vi "NumIntegrate_Rk4_Mat_X.vi"(5 "Func_X_Extra":refnum<vi>, 7 "PassedData":variant, 8 "dT_Seconds":dbl, 11 "X":T1) -> (0 "Error":bool, 3 "OUTPUT":T1)   [LabVIEW 2019, in "Trajectory_Library.lvlib"]
doc: "Performs 4th order Runge-Kutta integration of dx/dt = f( matrix x) for dt.\n\nInputs:\n - Func_X_Extra -- A strictly typed LabVIEW reference to a function to integrate as a function of matrix X, and the extra passed data\n - PassedData -- This is a variant that can be used to pass additional data to the function if needed. The data must be packed into the variant in the specific way expected by the function.\n - X -- X input matrix\n - dT -- Time differential in seconds\n\nOutputs:\n - OUTPUT -- The integration of dx/dt = f(x, u) for dt.\n - Error -- If TRUE, an error occured."
uses:
  Trajectory_Library.lvlib
  <vilib>/Analysis/Matrix/Datatypes/RealMatrix.ctl
  <vilib>/Analysis/Matrix/Numeric/Multiply/Multiply - RM,R.vi
  <vilib>/Analysis/Matrix/Numeric/Add/Add - RM,RM.vi
  <vilib>/Analysis/Matrix/NI_Matrix.lvlib
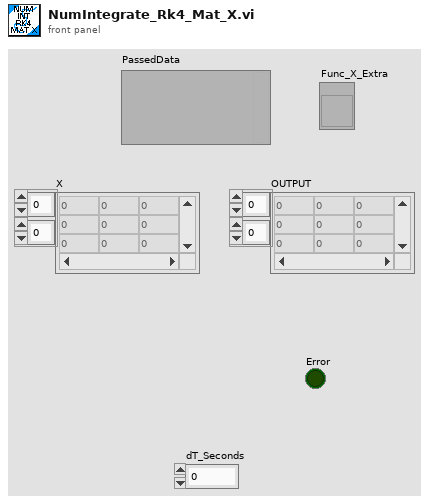
[diagram p1: front panel]
types:
  T1 = typedef "NI_Matrix.lvlib/RealMatrix.ctl" = dbl[][]
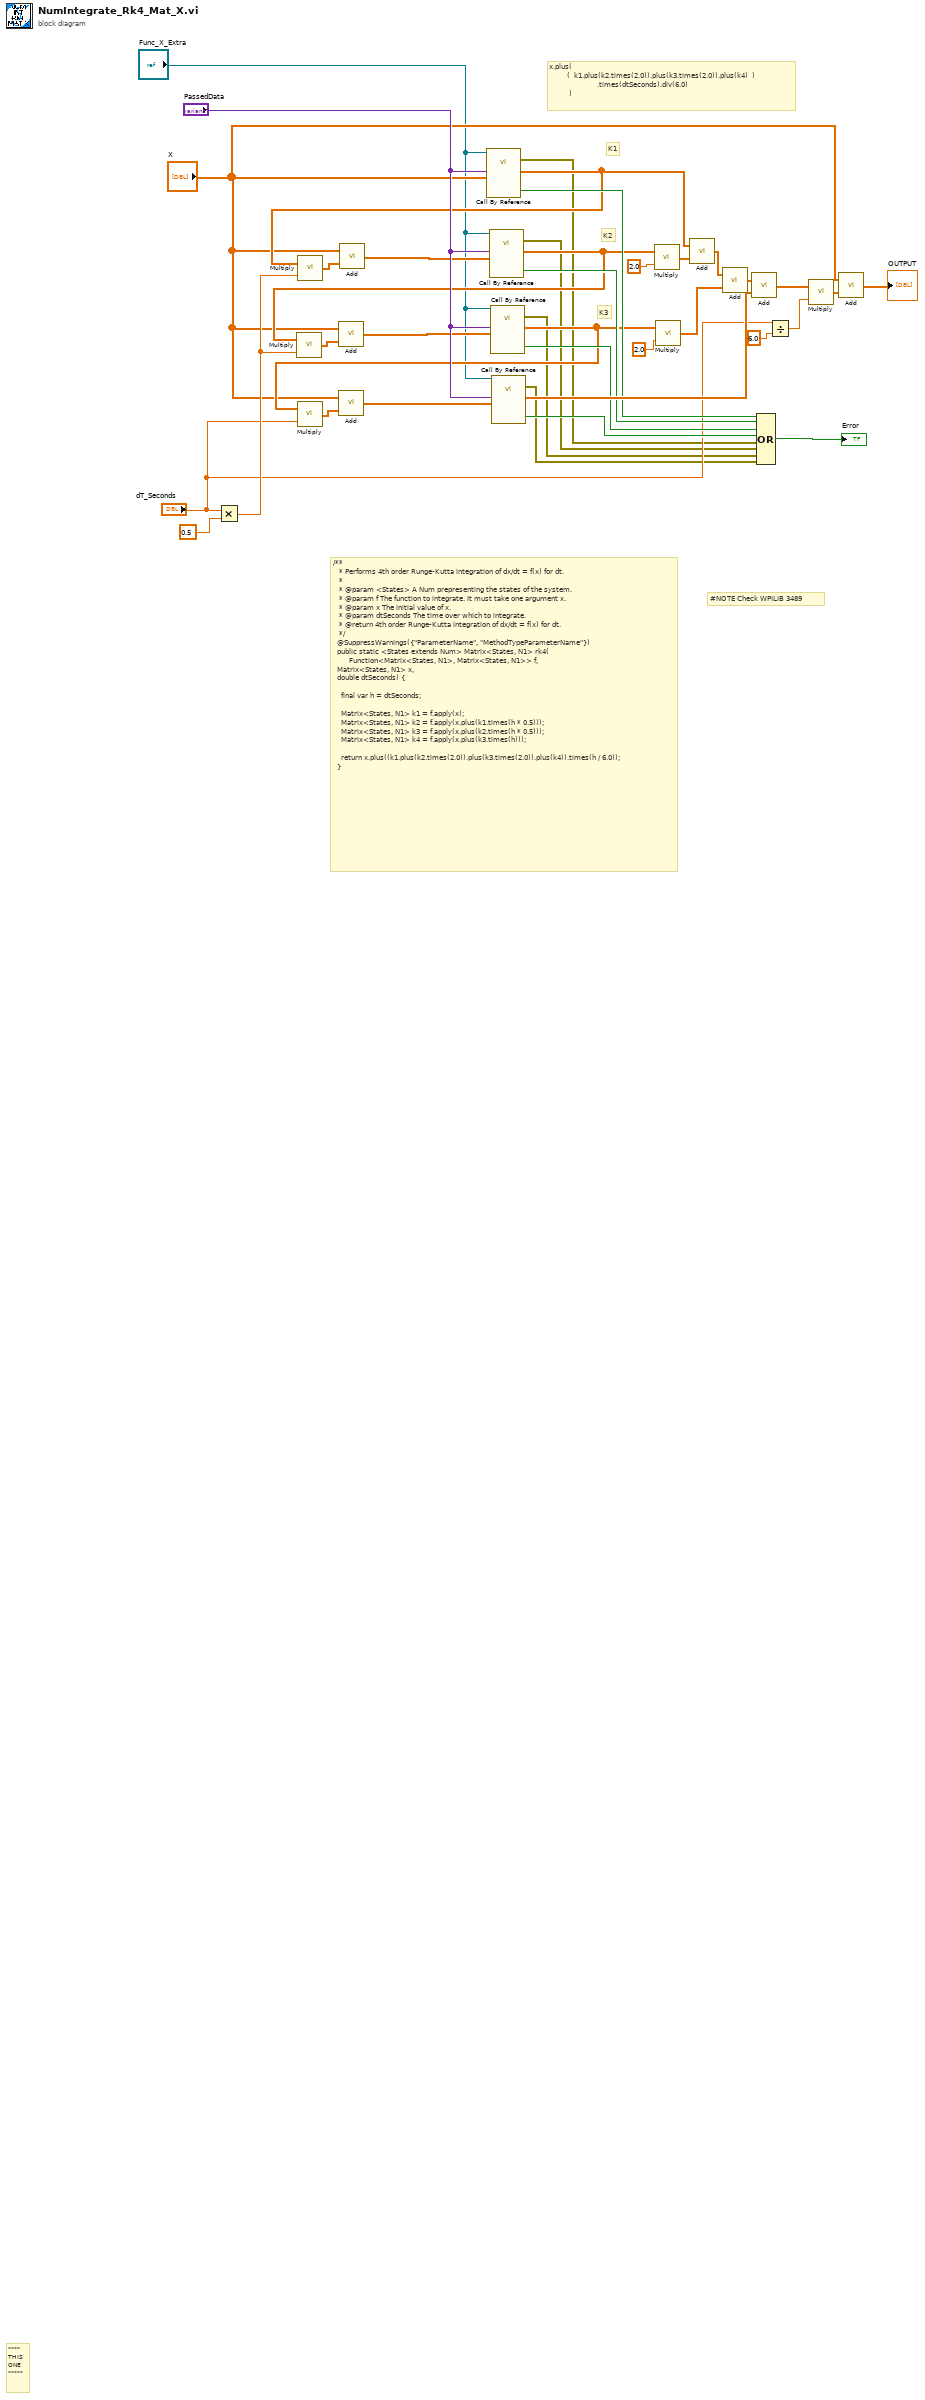
[diagram p0: block diagram]
diagram:
  # "#NOTE Check WPILIB 3489"
  # "x.plus(\n         (  k1.plus(k2.times(2.0)).plus(k3.times(2.0)).plus(k4)  )\n                        .times(dtSeconds).div(6.0)\n          )"
  # "K3"
  # "K2"
  # "K1"
  # "/**\n   * Performs 4th order Runge-Kutta integration of dx/dt = f(x) for dt.\n   *\n   * @param <States> A Num prepresenting the states of the system.\n   * @param f The function to integrate. It must take one argument x.\n   * @param x The initial value of x.\n   * @param dtSeconds The time over which to integrate.\n   * @return 4th order Runge-Kutta integration of dx/dt = f(x) for dt.\n   */\n  @SuppressWarnings({\"ParameterName\", \"MethodTypeParameterName\"})\n  public static <States extends Num> Matrix<States, N1> rk4(\n      \t\tFunction<Matrix<States, N1>, Matrix<States, N1>> f, \n\t\tMatrix<States, N1> x, \n\t\tdouble dtSeconds) {\n\n    final var h = dtSeconds;\n\n    Matrix<States, N1> k1 = f.apply(x);\n    Matrix<States, N1> k2 = f.apply(x.plus(k1.times(h * 0.5)));\n    Matrix<States, N1> k3 = f.apply(x.plus(k2.times(h * 0.5)));\n    Matrix<States, N1> k4 = f.apply(x.plus(k3.times(h)));\n\n    return x.plus((k1.plus(k2.times(2.0)).plus(k3.times(2.0)).plus(k4)).times(h / 6.0));\n  }"
  # "****\nTHIS\nONE\n*****"
  n1 = Multiply(x="dT_Seconds", y=0.5) -> (x*y=w13:dbl)
  n2 = call-by-ref "?"(reference="Func_X_Extra", "X"="X", "Variant"="PassedData") -> (error out=w5:errorcluster, "Error"=w28:bool, "NewX"=w22:T1)  [unwired: 9 in, 1 out]
  n3 = call-poly <vilib>:"Multiply.vi"("Real Scalar c"=w13, "Real Matrix A"=w22) -> ("A * c"=w21:T1)
  n4 = call-poly <vilib>:"Add.vi"("Real Matrix B"=w21, "Real Matrix A"="X") -> ("A + B"=w20:T1)
  n5 = call-by-ref "?"(reference="Func_X_Extra", "X"=w20, "Variant"="PassedData") -> (error out=w4:errorcluster, "Error"=w27:bool, "NewX"=w17:T1)  [unwired: 9 in, 1 out]
  n6 = call-poly <vilib>:"Multiply.vi"("Real Scalar c"=w13, "Real Matrix A"=w17) -> ("A * c"=w19:T1)
  n7 = call-poly <vilib>:"Add.vi"("Real Matrix B"=w19, "Real Matrix A"="X") -> ("A + B"=w18:T1)
  n8 = call-by-ref "?"(reference="Func_X_Extra", "X"=w18, "Variant"="PassedData") -> (error out=w3:errorcluster, "Error"=w26:bool, "NewX"=w14:T1)  [unwired: 9 in, 1 out]
  n9 = call-poly <vilib>:"Multiply.vi"("Real Scalar c"="dT_Seconds", "Real Matrix A"=w14) -> ("A * c"=w16:T1)
  n10 = call-poly <vilib>:"Add.vi"("Real Matrix B"=w16, "Real Matrix A"="X") -> ("A + B"=w15:T1)
  n11 = call-by-ref "?"(reference="Func_X_Extra", "X"=w15, "Variant"="PassedData") -> (error out=w2:errorcluster, "Error"=w25:bool, "NewX"=w29:T1)  [unwired: 9 in, 1 out]
  n12 = call-poly <vilib>:"Multiply.vi"("Real Scalar c"=2.0, "Real Matrix A"=w17) -> ("A * c"=w33:T1)
  n13 = call-poly <vilib>:"Multiply.vi"("Real Scalar c"=2.0, "Real Matrix A"=w14) -> ("A * c"=w31:T1)
  n14 = call-poly <vilib>:"Add.vi"("Real Matrix B"=w33, "Real Matrix A"=w22) -> ("A + B"=w32:T1)
  n15 = call-poly <vilib>:"Add.vi"("Real Matrix B"=w31, "Real Matrix A"=w32) -> ("A + B"=w30:T1)
  n16 = call-poly <vilib>:"Add.vi"("Real Matrix B"=w29, "Real Matrix A"=w30) -> ("A + B"=w12:T1)
  n17 = Compound Arithmetic op=OR(w28, w27, w26, w25, w5, w4, w3, w2) -> (→"Error":bool)
  n18 = Divide(x="dT_Seconds", y=6.0) -> (x/y=w9:dbl)
  n19 = call-poly <vilib>:"Multiply.vi"("Real Scalar c"=w9, "Real Matrix A"=w12) -> ("A * c"=w8:T1)
  n20 = call-poly <vilib>:"Add.vi"("Real Matrix B"=w8, "Real Matrix A"="X") -> ("A + B"=→"OUTPUT":T1)
